vi "New Execution.vi"(8 "error in (no error)":errorcluster, 10 "Execution Options":T1, 11 "Engine in":refnum<class "Engine.lvclass">) -> (0 "error out":errorcluster, 2 "Execution":refnum<class "Execution.lvclass">, 3 "Engine out":refnum<class "Engine.lvclass">)   [LabVIEW 2020, in "TSnax.lvlib" / "Engine.lvclass"]
uses:
  Engine.lvclass
  Execution Options.ctl
  Execution/Execution.lvclass
  Engine.lvclass/Engine.ctl
  TSnax.lvlib
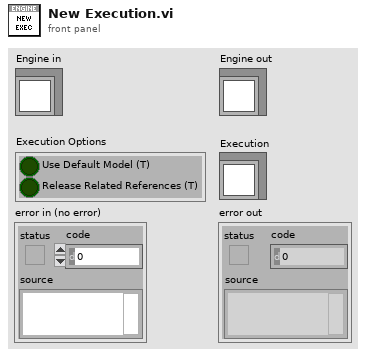
[diagram p1: front panel]
types:
  T1 = typedef "TSnax.lvlib/Execution Options.ctl" = cluster{"Use Default Model (T)":bool, "Release Related References (T)":bool}
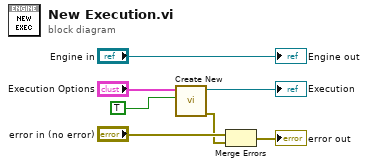
[diagram p0: block diagram]
diagram:
  n1 = call "Create New.vi"("Daemonized"=TRUE, "Options"="Execution Options") -> ("error out"=w2:errorcluster, "Execution out"=→"Execution":refnum<class "Execution.lvclass">)  [unwired: 8 in]
  n2 = Merge Errors("error in (no error)", w2) -> (→"error out":errorcluster)
  "Engine out" <- "Engine in"
